vi "Is Index In Range (1D Array).vi"(1 "Index":i32, 2 "Array Number of Elements (Array Size)":i32) -> (0 "Is Index In Range?":bool)   [LabVIEW 2026, in "RSysUtils Array.lvlib"]
doc: "This VI checks whether the Index is inside the Range (the number of elements) of an Array.\nThis VI outputs True if and only if the \"Index\" has a value between 0 and \"Array Number of Elements - 1\".\nThis VI outputs False if \"Array Number of Elements\" <= 0."
uses:
  RSysUtils Array.lvlib
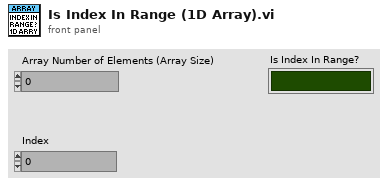
[diagram p1: front panel]
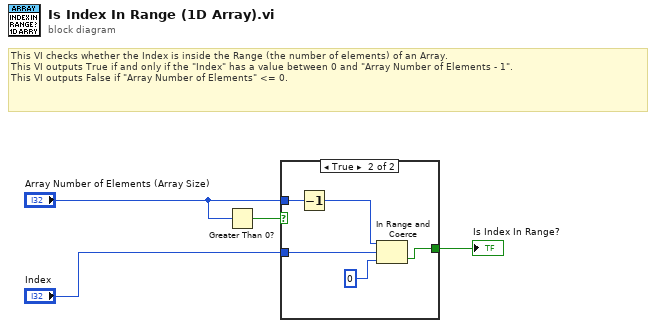
[diagram p0: block diagram]
diagram:
  # "This VI checks whether the Index is inside the Range (the number of elements) of an Array.\nThis VI outputs True if and only if the \"Index\" has a value between 0 and \"Array Number of Elements - 1\".\nThis VI outputs False if \"Array Number of Elements\" <= 0."
  n1 = Greater Than 0?(x="Array Number of Elements (Array Size)") -> (x > 0?=w2:bool)
  n2 = case shown="True" w2 {
    tunnel: [_ w9] -> w4
    tunnel: "Array Number of Elements (Array Size)" -> [_ w8]
    tunnel: "Index" -> [_ w5]
    frame False {
    }
    frame True {
      n3 = Decrement(x=w8) -> (x-1=w7:i32)
      n4 = In Range and Coerce(upper limit=w7, x=w5, lower limit=0) -> (In Range?=w9:bool)  [unwired: 1 out]
    }
  }
  "Is Index In Range?" <- w4
